vi "Add Controller.vi"(8 "error in":errorcluster, 10 "IController":refnum<class "IController.lvclass">, 11 "Cell in":refnum<class "Cell.lvclass">) -> (0 "error out":errorcluster, 3 "Cell out":refnum<class "Cell.lvclass">)   [LabVIEW 2020, in "SourceGrid.lvlib" / "Cell.lvclass"]
uses:
  Cell.lvclass
  Controllers/IController/IController.lvclass
  Cell.lvclass/Cell.ctl
  D:/git/Sourcegrid-LabVIEW/source/SourceGrid.dll
  SourceGrid.dll
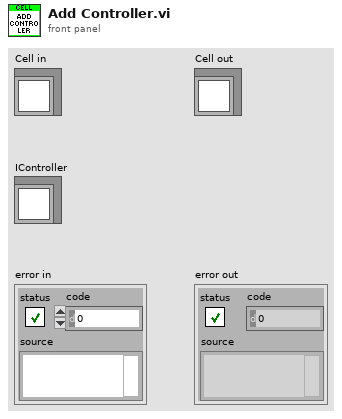
[diagram p1: front panel]
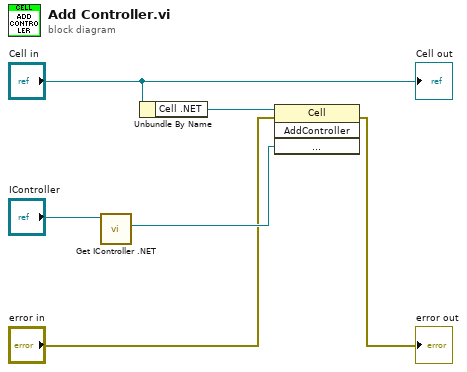
[diagram p0: block diagram]
diagram:
  n1 = call-dynamic "Get IController .NET.vi"("IController in"="IController") -> ("IController"=w3:refnum<k24>)  [unwired: 9 in, 1 out]
  n2 = Unbundle By Name("Cell in") -> ("Cell .NET"=w5:refnum<k24>)
  n3 = invoke class="Cell" method="AddController"(reference=w5, error in="error in", "controller"=w3) -> (error out=→"error out":errorcluster)  [unwired: 1 in, 3 out]
  "Cell out" <- "Cell in"
